vi "get channels.vi"(11 "Shared Memory configuration in":refnum<class "Shared Memory configuration.lvclass">) -> (2 "channels":refnum<class "TBM channel.lvclass">[](array[class]), 3 "Shared Memory configuration out":refnum<class "Shared Memory configuration.lvclass">)   [LabVIEW 2014, in "Shared Memory configuration.lvclass"]
doc: "Returns an array of all Channels currently added to this configuration object."
uses:
  Shared Memory configuration.lvclass
  <vilib>/NI/Tag Bus Module Framework/channel/TBM channel.lvclass
  Shared Memory configuration.lvclass/Shared Memory configuration.ctl
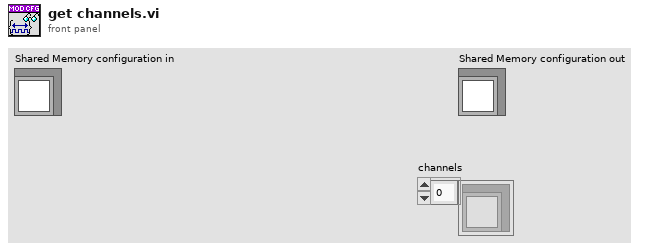
[diagram p1: front panel]
types:
  T1 = typedef "Shared Memory configuration.lvclass/Line.ctl" = cluster{"channel":refnum<class "TBM channel.lvclass">}
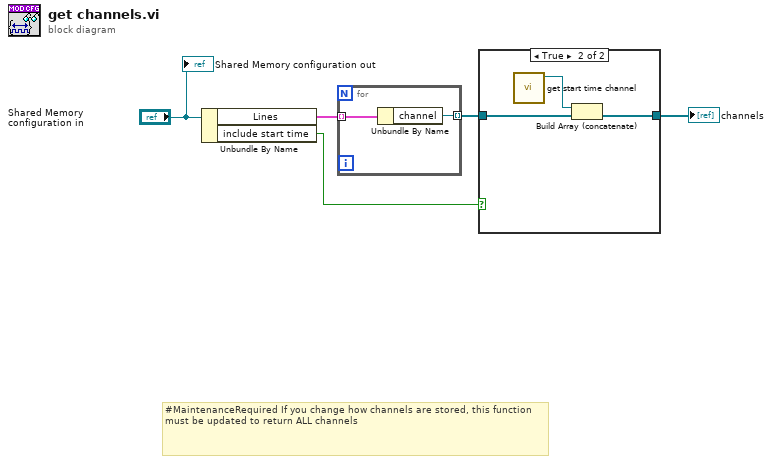
[diagram p0: block diagram]
diagram:
  # "#MaintenanceRequired If you change how channels are stored, this function must be updated to return ALL channels"
  n1 = Unbundle By Name("Shared Memory configuration in") -> ("Lines"=w4:T1[], "include start time"=w3:bool)
  n2 = for {
    tunnel: w4 -> [w7] mode=indexing
    tunnel: [w6] -> w2 mode=indexing
    n3 = Unbundle By Name(w7) -> ("channel"=w6:refnum<class "TBM channel.lvclass">)
  }
  n4 = case shown="True" w3 {
    tunnel: w2 -> [w8 w10]
    tunnel: [w8 w9] -> w1
    frame False {
    }
    frame True {
      n5 = call "get start time channel.vi"() -> ("channel"=w11:refnum<class "TBM channel.lvclass">)  [unwired: 11 in]
      n6 = Build Array (concatenate)(w11, w10) -> (w9:refnum<class "TBM channel.lvclass">[])
    }
  }
  "channels" <- w1
  "Shared Memory configuration out" <- "Shared Memory configuration in"
